vi "Route Switch Box Command.vi"(8 "error in (no error)":errorcluster caption="에러 입력(에러 없음)", 10 "문자열":string, 11 "Instrument Manager 입력":refnum<class "Instrument Manager.lvclass">) -> (0 "error out":errorcluster caption="에러 출력", 3 "Instrument Manager 출력":refnum<class "Instrument Manager.lvclass">)   [LabVIEW 2023, in "Instrument Manager.lvclass"]
uses:
  Instrument Manager.lvclass
  <vilib>/regexp/Match Regular Expression.xnode
  Instrument Manager.lvclass/Instrument Manager.ctl
panel:
  out "Ip Info":cluster{"ip address":string, "port":u16}
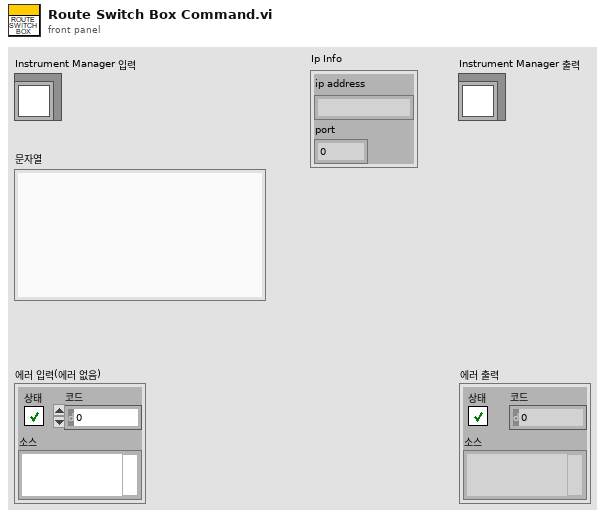
[diagram p1: front panel]
types:
  T1 = typedef "Instrument Manager.lvclass/Connect Switch Box Param.ctl" = cluster{"type":string, "id":string, "target":string, "command":string, "Params":cluster{"ip address":string, "port":i32}}
  T2 = typedef "RF Switch Box.lvlib/Input path.ctl" = enum16{"Input 1", "Input 2", "Input 3"}
  T3 = typedef "Instrument Manager.lvclass/Set Input Path Param.ctl" = cluster{"type":string, "id":string, "target":string, "command":string, "Params":cluster{"Input Path":i32}}
  T4 = typedef "RF Switch Box.lvlib/Filter path.ctl" = enum16{"Thru", "Direct Amp", "1G HPF", "3G HPF", "7G HPF", "6G HPF", "port 1", "port 2", "port 3", "port 4", "port 5", "port 6", "port 7", "port 8", "port 9", "port 10", "port 11", "port 12", "port 13", "port 14", "port 15", "port 16", "port 17", "port 18"}
  T5 = typedef "Instrument Manager.lvclass/Set Filter Path Param.ctl" = cluster{"type":string, "id":string, "target":string, "command":string, "Params":cluster{"Filter Path":i32}}
  T6 = typedef "Instrument Manager.lvclass/Set Path Param.ctl" = cluster{"type":string, "id":string, "target":string, "command":string, "Params":cluster{"Input Path":i32, "Filter Path":i32}}
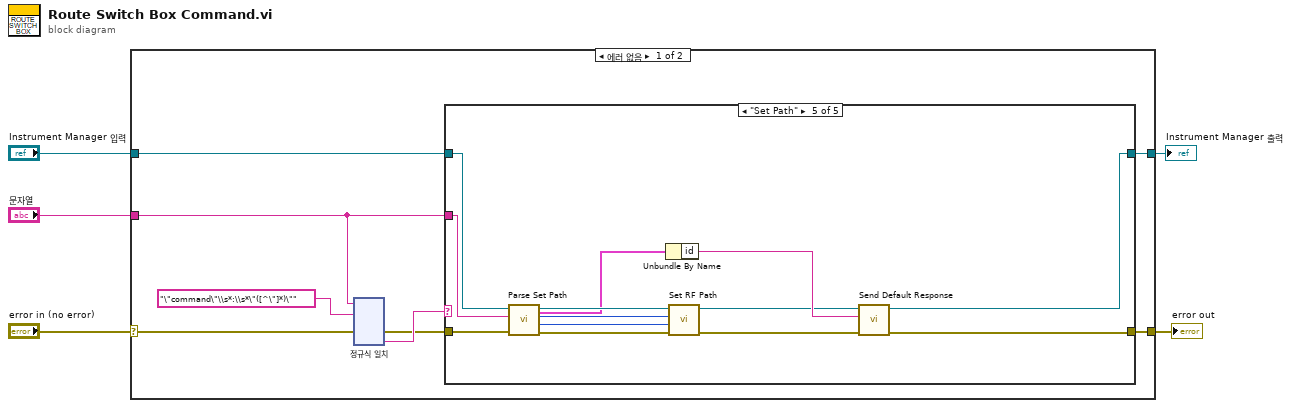
[diagram p0: block diagram]
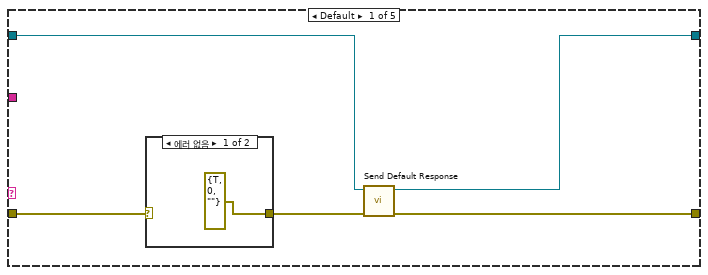
[diagram p2: hidden frame]
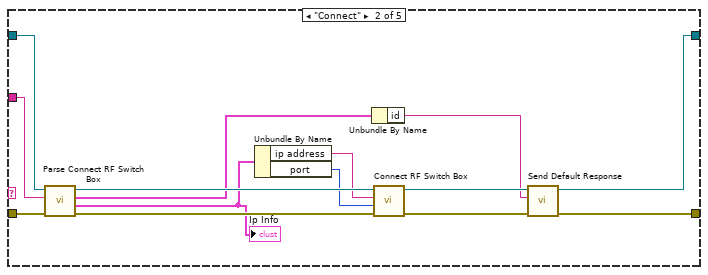
[diagram p4: hidden frame]
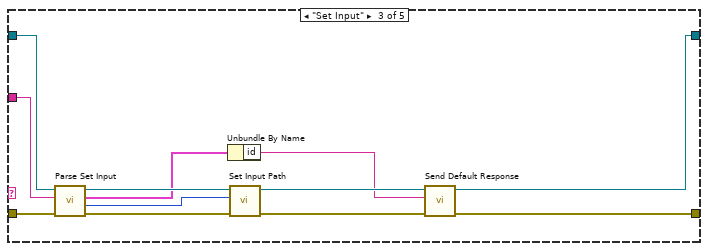
[diagram p5: hidden frame]
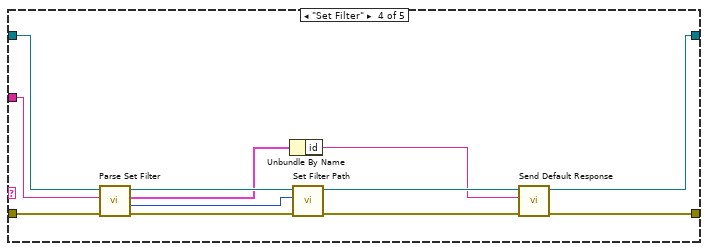
[diagram p6: hidden frame]
diagram:
  n1 = case shown="에러 없음" "error in (no error)" {
    selector: "error in (no error)" -> [w6 w192]
    tunnel: [w8 w192] -> w4
    tunnel: [w7 w191] -> w2
    tunnel: "Instrument Manager 입력" -> [w9 w191]
    tunnel: "문자열" -> [w10 _]
    frame No Error {
      n2 = xnode "정규식 일치"("입력 문자열"=w10, "정규식"="\"command\"\\s*:\\s*\"([^\"]*)\"", "에러 입력"=w6) -> ("에러 출력"=w11:errorcluster, "부분 일치 1"=w12:string)  [unwired: 3 in, 4 out]
      n3 = case shown="\"Set Path\"" w12 {
        tunnel: w11 -> [w17 w34 w44 w56 w61]
        tunnel: w10 -> [_ w27 w45 w57 w63]
        tunnel: w9 -> [w15 w30 w46 w58 w62]
        tunnel: [w16 w31 w40 w53 w60] -> w8
        tunnel: [w14 w25 w37 w47 w59] -> w7
        frame Default {
          n4 = case shown="에러 없음" w17 {
            selector: w17 -> [_ w20]
            tunnel: [errorcluster {"status"=TRUE, "code"=0, "source"=""} ("error IO") w20] -> w18
            frame No Error {
            }
            frame Error {
            }
          }
          n5 = call "Send Default Response.vi"("error in (no error)"=w18, "Instrument Manager 입력"=w15) -> ("error out"=w16:errorcluster, "Instrument Manager 출력"=w14:refnum<class "Instrument Manager.lvclass">)  [unwired: 8 in]
        }
        frame "Connect" {
          n6 = call "Parse Connect RF Switch Box.vi"("error in (no error)"=w34, "JSON string"=w27, "Instrument Manager 입력"=w30) -> ("error out"=w33:errorcluster, "Ip Info"=w21:cluster{"ip address":string, "port":u16}, "Connect Switch Box Param"=w26:T1, "Instrument Manager 출력"=w29:refnum<class "Instrument Manager.lvclass">)  [unwired: 5 in]
          "Ip Info" <- w21
          n7 = Unbundle By Name(w21) -> ("ip address"=w23:string, "port"=w22:u16)
          n8 = Unbundle By Name(w26) -> ("id"=w24:string)
          n9 = call "Connect RF Switch Box.vi"("error in (no error)"=w33, "포트"=w22, "주소"=w23, "Instrument Manager 입력"=w29) -> ("error out"=w32:errorcluster, "Instrument Manager 출력"=w28:refnum<class "Instrument Manager.lvclass">)  [unwired: 6 in]
          n10 = call "Send Default Response.vi"("error in (no error)"=w32, "id"=w24, "Instrument Manager 입력"=w28) -> ("error out"=w31:errorcluster, "Instrument Manager 출력"=w25:refnum<class "Instrument Manager.lvclass">)  [unwired: 7 in]
        }
        frame "Set Input" {
          n11 = call "Parse Set Input.vi"("error in (no error)"=w44, "JSON string"=w45, "Instrument Manager 입력"=w46) -> ("error out"=w42:errorcluster, "Input path"=w43:T2, "Set Input Param"=w36:T3, "Instrument Manager 출력"=w39:refnum<class "Instrument Manager.lvclass">)  [unwired: 4 in]
          n12 = Unbundle By Name(w36) -> ("id"=w35:string)
          n13 = call "Set Input Path.vi"("error in (no error)"=w42, "Input path"=w43, "Instrument Manager 입력"=w39) -> ("error out"=w41:errorcluster, "Instrument Manager 출력"=w38:refnum<class "Instrument Manager.lvclass">)  [unwired: 7 in]
          n14 = call "Send Default Response.vi"("error in (no error)"=w41, "id"=w35, "Instrument Manager 입력"=w38) -> ("error out"=w40:errorcluster, "Instrument Manager 출력"=w37:refnum<class "Instrument Manager.lvclass">)  [unwired: 7 in]
        }
        frame "Set Filter" {
          n15 = call "Parse Set Filter.vi"("error in (no error)"=w56, "JSON string"=w57, "Instrument Manager 입력"=w58) -> ("error out"=w55:errorcluster, "Filter path"=w50:T4, "Set Filter Param"=w49:T5, "Instrument Manager 출력"=w52:refnum<class "Instrument Manager.lvclass">)  [unwired: 5 in]
          n16 = Unbundle By Name(w49) -> ("id"=w48:string)
          n17 = call "Set Filter Path.vi"("error in (no error)"=w55, "Filter path"=w50, "Instrument Manager 입력"=w52) -> ("error out"=w54:errorcluster, "Instrument Manager 출력"=w51:refnum<class "Instrument Manager.lvclass">)  [unwired: 7 in]
          n18 = call "Send Default Response.vi"("error in (no error)"=w54, "id"=w48, "Instrument Manager 입력"=w51) -> ("error out"=w53:errorcluster, "Instrument Manager 출력"=w47:refnum<class "Instrument Manager.lvclass">)  [unwired: 7 in]
        }
        frame "Set Path" {
          n19 = call "Parse Set Path.vi"("error in (no error)"=w61, "JSON string"=w63, "Instrument Manager 입력"=w62) -> ("error out"=w69:errorcluster, "Filter path"=w70:T4, "Input path"=w71:T2, "Instrument Manager 출력"=w68:refnum<class "Instrument Manager.lvclass">, "Set Path Param"=w67:T6)  [unwired: 4 in]
          n20 = Unbundle By Name(w67) -> ("id"=w65:string)
          n21 = call "Set RF Path.vi"("error in (no error)"=w69, "Filter path"=w70, "Input path"=w71, "Instrument Manager 입력"=w68) -> ("error out"=w66:errorcluster, "Instrument Manager 출력"=w64:refnum<class "Instrument Manager.lvclass">)  [unwired: 6 in]
          n22 = call "Send Default Response.vi"("error in (no error)"=w66, "id"=w65, "Instrument Manager 입력"=w64) -> ("error out"=w60:errorcluster, "Instrument Manager 출력"=w59:refnum<class "Instrument Manager.lvclass">)  [unwired: 7 in]
        }
      }
    }
    frame Error {
    }
  }
  "error out" <- w4
  "Instrument Manager 출력" <- w2
